vi "Initialize Scalar Datatypes and Refs.vi"(8 "error in (no error)":errorcluster, 9 "session in":u32, 10 "Registers":T1[](array[typedef]) {"Register"."Data Type" format="%.0x"}) -> (0 "error out":errorcluster, 1 "session out":u32, 2 "Registers Ref":T5[](array[typedef]) {"Data Type" format="%.0x"})   [LabVIEW 2020, in "FPGA Addon Engine.lvlib"]
uses:
  FPGA Addon Engine.lvlib
  Types/Register Settings.ctl
  Addon Shared/Types/Scalar Type.ctl
  Addon Shared/FPGA Addon Shared.lvlib
  Addon Shared/Types/Register Information.ctl
  Addon Shared/Types/Compiled.RegisterSettings.ctl
  Addon Shared/Types/FPGA Addon Data Type.ctl
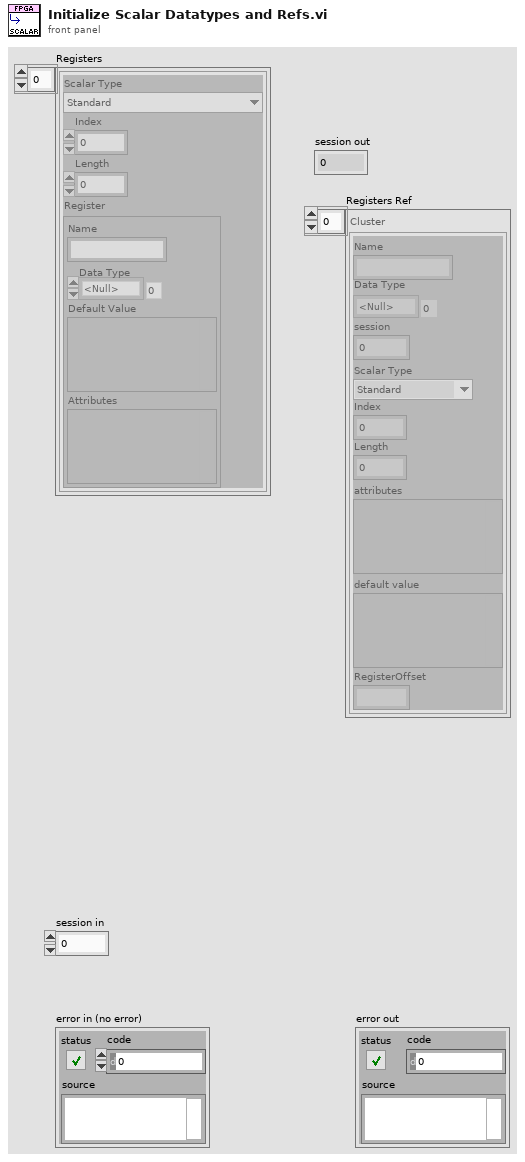
[diagram p1: front panel]
types:
  T1 = typedef "FPGA Addon Shared.lvlib/Compiled.RegisterSettings.ctl" = cluster{"Scalar Type":T2, "Index":i32, "Length":i32, "Register":T3}
  T2 = typedef "FPGA Addon Shared.lvlib/Scalar Type.ctl" = enum16{"Standard", "Bitpacked"}
  T3 = typedef "FPGA Addon Shared.lvlib/Register Information.ctl" = cluster{"Name":string, "Data Type":T4, "Default Value":variant, "Attributes":variant}
  T4 = typedef "FPGA Addon Shared.lvlib/FPGA Addon Data Type.ctl" = enum8{"<Null>", "I8", "I16", "I32", "I64", "U8", "U16", "U32", "U64", "SGL", "Boolean", "Analog PWM In Settings", "Analog PWM In", "Digital PWM In Settings", "Digital PWM In", "Digital PWM Out", "Sine Out", "FXP", "FXP+/-24.5", "FXP+/-16.5", "FXP+/-32.8", "FXP+/-64.32", "FXP+/-16.7", "FXP+/-20.5", "FXP+/-27.5", "FXP+/-32.16", "FXP+16.3", "FXP+18.3", "Digital Static In", "Digital Static Out", "Digital Static In Settings", "Digital WSS Out", "Quad Encoder Settings", "Quad Encoder In", "Group"}
  T5 = typedef "FPGA Addon Engine.lvlib/Register Settings.ctl" = cluster{"Name":string, "Data Type":T4, "session":u32, "Scalar Type":T2, "Index":i32, "Length":i32, "attributes":variant, "default value":variant, "RegisterOffset":u32}
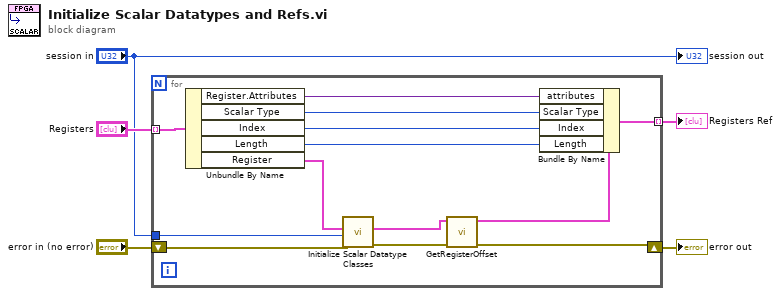
[diagram p0: block diagram]
diagram:
  n1 = for {
    tunnel: [w18] -> w5 mode=indexing
    tunnel: "Registers" -> [w17] mode=indexing
    shift-right: [w6] -> w3
    shift-left: "error in (no error)" -> [w12]
    tunnel: "session in" -> [w10]
    n2 = Unbundle By Name(w17) -> ("Register.Attributes"=w11:variant, "Scalar Type"=w13:T2, "Index"=w14:i32, "Length"=w15:i32, "Register"=w16:T3)
    n3 = call "Initialize Scalar Datatype Classes.vi"("error in (no error)"=w12, "session in"=w10, "Register"=w16) -> ("error out"=w9:errorcluster, "Register"=w8:T5)  [unwired: 7 in]
    n4 = call "GetRegisterOffset.vi"("error in (no error)"=w9, "element in"=w8) -> ("error out"=w6:errorcluster, "element out"=w7:T5)  [unwired: 7 in, 1 out]
    n5 = Bundle By Name(cluster=w7, "attributes"=w11, "Scalar Type"=w13, "Index"=w14, "Length"=w15) -> (w18:T5)
  }
  "error out" <- w3
  "Registers Ref" <- w5
  "session out" <- "session in"
